vi "Send Data for UI.vi"(0 "Measure Call Context in":refnum<class "Measure Call Context.lvclass">, 1 "fpga interface in":refnum<k20>, 2 "Embedded Data":T2, 3 "Last displayed image data":u32[](array[numeric]), 5 "FrameCount":u64, 7 "registers":string[][](array[string])=[["0x10", "0x2030", "0x01f0"], ["0x10", "0x3120", "0x0802"]], 9 "References":T4, 11 "error in":errorcluster, 12 "Status data":T6, 13 "SOURCE RATE (fps)":dbl, 14 "Active Channel":string) -> (4 "output cluster":T1={"ACQ. IN PROGRESS"=FALSE, "IMAGE PIXEL DATA"=[], "ACQ. DURATION (s)"=0.0, "SOURCE RATE (fps)"=0.0, "BYTES ACQUIRED"=0, "FRAME COUNT"=0, "POC VOLTAGE (V)"=0.0, "POC CURRENT (A)"=0.0, "ERROR"=FALSE, "STATE MESSAGE"="Initializing...", "IMAGE DATA"="", "OOB gRPC Port"=0, "HEIGHT"=0, "WIDTH"=0, "FRAME COUNT BYTES"=[], "REGISTERS"=[], "COUNT LENGTH"=0} {"BYTES ACQUIRED" format="%#.6p"}, 15 "error out":errorcluster)   [LabVIEW 2025, in "Automotive Vision.lvclass"]
doc: "Handles data transfer to the UI."
uses:
  Automotive Vision.lvclass
  <vilib>/Plug-In SDKs/Measurements/Measure Call Context/Measure Call Context.lvclass
  <instrlib>/FlexRIO/CSI-2/v2/Common/Types/LLP Data Type.ctl
  embedded data.ctl
  embedded data item.ctl
  Measurement Results.ctl
  Automotive Vision.lvclass/Automotive Vision.ctl
  <instrlib>/FlexRIO/CSI-2/v2/Common/NI CSI-2 API Common v2.lvlib
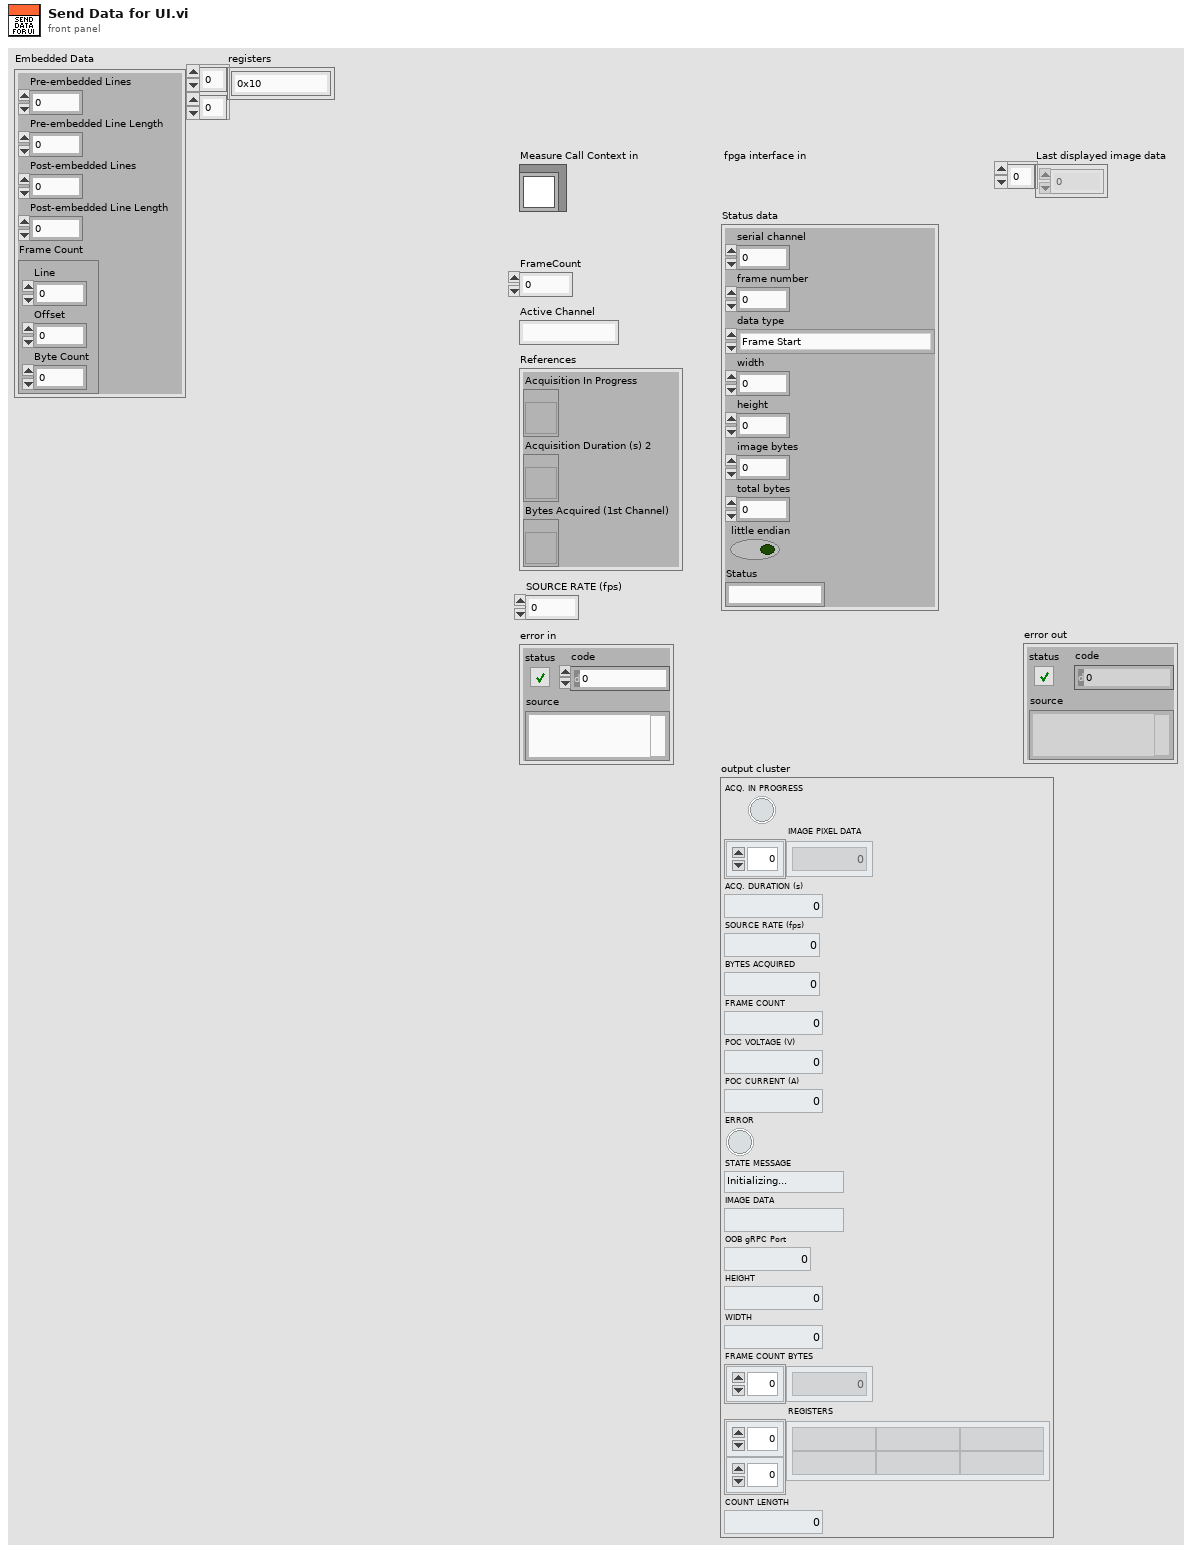
[diagram p1: front panel]
types:
  T1 = typedef "Automotive Vision.lvclass/Measurement Results.ctl" = cluster{"ACQ. IN PROGRESS":bool, "IMAGE PIXEL DATA":u32[], "ACQ. DURATION (s)":dbl, "SOURCE RATE (fps)":dbl, "BYTES ACQUIRED":u64, "FRAME COUNT":u64, "POC VOLTAGE (V)":dbl, "POC CURRENT (A)":dbl, "ERROR":bool, "STATE MESSAGE":string, "IMAGE DATA":string, "OOB gRPC Port":i32, "HEIGHT":u64, "WIDTH":u64, "FRAME COUNT BYTES":u32[], "REGISTERS":string[][], "COUNT LENGTH":u64}
  T2 = typedef "Automotive Vision.lvclass/embedded data.ctl" = cluster{"Pre-embedded Lines":dbl, "Pre-embedded Line Length":dbl, "Post-embedded Lines":dbl, "Post-embedded Line Length":dbl, "Frame Count":T3}
  T3 = typedef "Automotive Vision.lvclass/embedded data item.ctl" = cluster{"Line":dbl, "Offset":dbl, "Byte Count":dbl}
  T4 = cluster{"Acquisition In Progress":refnum<vi>, "Acquisition Duration (s) 2":refnum<vi>, "Bytes Acquired (1st Channel)":refnum<vi>}
  T5 = typedef "NI CSI-2 API Common v2.lvlib/LLP Data Type.ctl" = enum8{"Frame Start", "Frame End", "Line Start", "Line End", "End of Transmission", "Reserved 0", "Reserved 1", "Reserved 2", "Generic Short Packet 1", "Generic Short Packet 2", "Generic Short Packet 3", "Generic Short Packet 4", "Generic Short Packet 5", "Generic Short Packet 6", "Generic Short Packet 7", "Generic Short Packet 8", "Null", "Blanking Data", "Embedded 8-bit non Image Data", "Generic Long Packet 1", "Generic Long Packet 2", "Generic Long Packet 3", "Generic Long Packet 4", "Reserved 3", "YUV420 8-bit", "YUV420 10-bit", "Legacy YUV420 8-bit", "Reserved 4", "YUV420 8-bit Chroma Shifted", "YUV420 10-bit Chroma Shifted", "YUV422 8-bit", "YUV422 10-bit", "RGB444", "RGB555", "RGB565", "RGB666", "RGB888", "Reserved 5", "Reserved 6", "RAW 24", "RAW 6", "RAW 7", "RAW 8", "RAW 10", "RAW 12", "RAW 14", "RAW 16", "RAW 20", "User Defined 8-bit Data 1", "User Defined 8-bit Data 2", "User Defined 8-bit Data 3", "User Defined 8-bit Data 4", "User Defined 8-bit Data 5", "User Defined 8-bit Data 6", "User Defined 8-bit Data 7", "User Defined 8-bit Data 8", "USL Command", "Reserved 7", "Reserved 8", "Reserved 9", "Reserved 10", "Reserved 11", "Reserved 12", "LRTE EPD Spacer"}
  T6 = cluster{"serial channel":fxp<+,3,3>, "frame number":u16, "data type":T5, "width":u16, "height":u16, "image bytes":u32, "total bytes":u32, "little endian":bool, "Status":string}
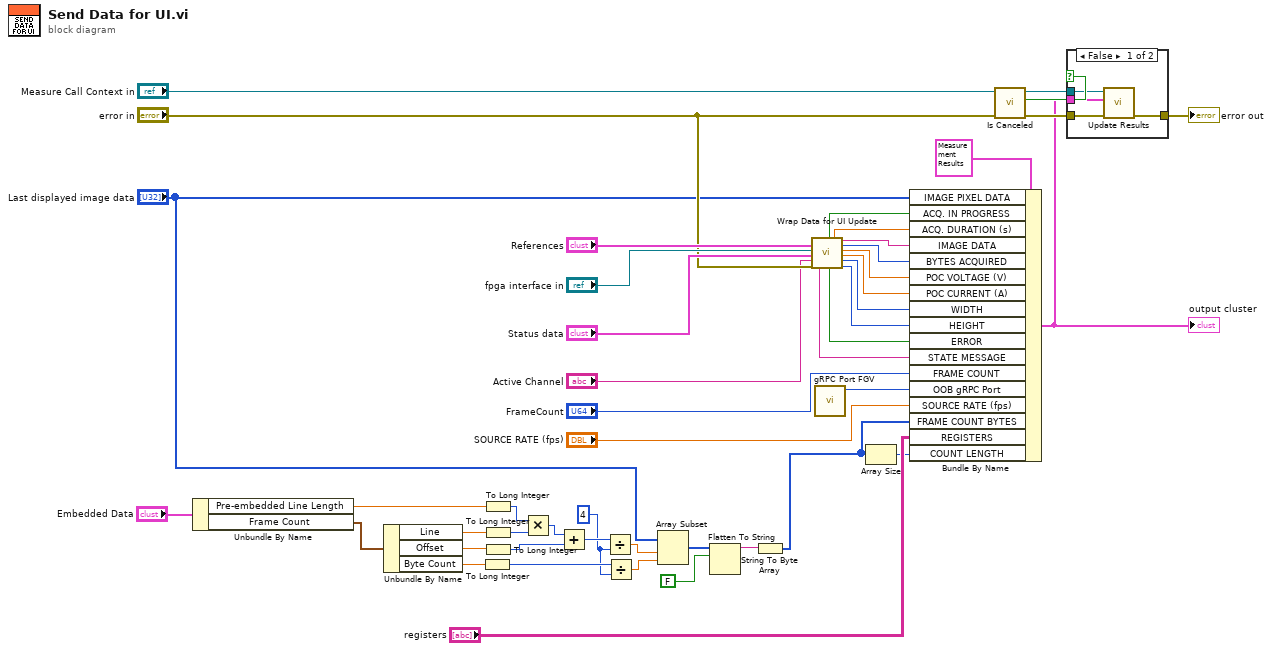
[diagram p0: block diagram]
diagram:
  w7 = 4 ("y")
  n1 = Unbundle By Name("Embedded Data") -> ("Pre-embedded Line Length"=w18:dbl, "Frame Count"=w22:T3)
  n2 = Unbundle By Name(w22) -> ("Line"=w16:dbl, "Offset"=w14:dbl, "Byte Count"=w12:dbl)
  n3 = To Long Integer(number=w12) -> (32bit integer=w8:i32)
  n4 = To Long Integer(number=w18) -> (32bit integer=w17:i32)
  n5 = To Long Integer(number=w16) -> (32bit integer=w15:i32)
  n6 = To Long Integer(number=w14) -> (32bit integer=w13:i32)
  n7 = Multiply(x=w17, y=w15) -> (x*y=w21:i32)
  n8 = Add(x=w21, y=w13) -> (x+y=w11:i32)
  n9 = Divide(x=w11, y=w7) -> (x/y=w10:dbl)
  n10 = Divide(x=w8, y=w7) -> (x/y=w9:dbl)
  n11 = Array Subset(array="Last displayed image data", index=w10, length=w9) -> (w4:u32[])
  n12 = Flatten To String(anything=w4, prepend array or string size? (T)=FALSE) -> (data string=w5:string)  [unwired: 2 in, 2 out]
  n13 = String To Byte Array(string=w5) -> (unsigned byte array=w1:u8[])
  n14 = call "Wrap Data for UI Update.vi"("References"="References", "fpga inteface in"="fpga interface in", "image metadata"="Status data", "Active Channel"="Active Channel", "error in"="error in") -> ("State message"=w37:string, "Acqusition In Progress"=w32:bool, "status"=w36:bool, "Acquisition Duration"=w33:dbl, "Image Data"=w27:string, "Bytes Acquired"=w28:u64, "PowerOverCoaxCurrent"=w34:dbl, "PowerOverCoaxVoltage"=w35:dbl, "width"=w45:u64, "height"=w46:u64)  [unwired: 5 in]
  n15 = call "gRPC Port FGV.vi"() -> ("Listening Port out"=w44:i32)  [unwired: 11 in]
  n16 = Array Size(array=w1) -> (size(s)=w19:i32)
  n17 = Bundle By Name(cluster=T1 {"ACQ. IN PROGRESS"=FALSE, "IMAGE PIXEL DATA"=[], "ACQ. DURATION (s)"=0.0, "SOURCE RATE (fps)"=0.0, "BYTES ACQUIRED"=0, "FRAME COUNT"=0, "POC VOLTAGE (V)"=0.0, "POC CURRENT (A)"=0.0, "ERROR"=FALSE, "STATE MESSAGE"="", "IMAGE DATA"="", "OOB gRPC Port"=0, "HEIGHT"=0, "WIDTH"=0, "FRAME COUNT BYTES"=[], "REGISTERS"=[], "COUNT LENGTH"=0} ("Measurement Results"), "IMAGE PIXEL DATA"="Last displayed image data", "ACQ. IN PROGRESS"=w32, "ACQ. DURATION (s)"=w33, "IMAGE DATA"=w27, "BYTES ACQUIRED"=w28, "POC VOLTAGE (V)"=w34, "POC CURRENT (A)"=w35, "WIDTH"=w45, "HEIGHT"=w46, "ERROR"=w36, "STATE MESSAGE"=w37, "FRAME COUNT"="FrameCount", "OOB gRPC Port"=w44, "SOURCE RATE (fps)"="SOURCE RATE (fps)", "FRAME COUNT BYTES"=w1, "REGISTERS"="registers", "COUNT LENGTH"=w19) -> (w30:T1)
  "output cluster" <- w30
  n18 = call <vilib>:"Is Canceled.vi"("error in"="error in", "measure call context in"="Measure Call Context in") -> ("error out"=w43:errorcluster, "is canceled?"=w42:bool, "measure call context out"=w41:refnum<class "Measure Call Context.lvclass">)  [unwired: 7 in]
  n19 = case shown="False" w42 {
    tunnel: w30 -> [w51 _]
    tunnel: [w50 w52] -> w31
    tunnel: w41 -> [w49 _]
    tunnel: w43 -> [w48 w52]
    frame False {
      n20 = call <vilib>:"Update Results.vi"("error in"=w48, "measurement results"=w51, "measure call context in"=w49) -> ("error out"=w50:errorcluster)  [unwired: 7 in, 1 out]
    }
    frame True {
    }
  }
  "error out" <- w31
